vi "test_lidar3.vi"() -> ()   [LabVIEW 2017]
panel:
  out "subarray 2":dbl[][](array[numeric])
  out "subarray 1":dbl[][](array[numeric])
  out "Boucle 2":bool
  out "Boucle 1":bool
  out "output array":dbl[][](array[numeric])
  in  "Array":dbl[][](array[numeric])=[[0.0, 1.0, 2.0, 3.0, 4.0, 355.0, 356.0, 357.0, 358.0, 359.0], [26.0, 12.0, 15.0, 32.0, 27.0, 22.0, 11.0, 23.0, 51.0, 16.0], [0.0, 0.0, 0.0, 0.0, 0.0, 0.0, 0.0, 0.0, 0.0, 0.0]]
  out "Div":dbl
  in  "Alpha 2":i32=8
  out "Nbr a enlever 2":i32
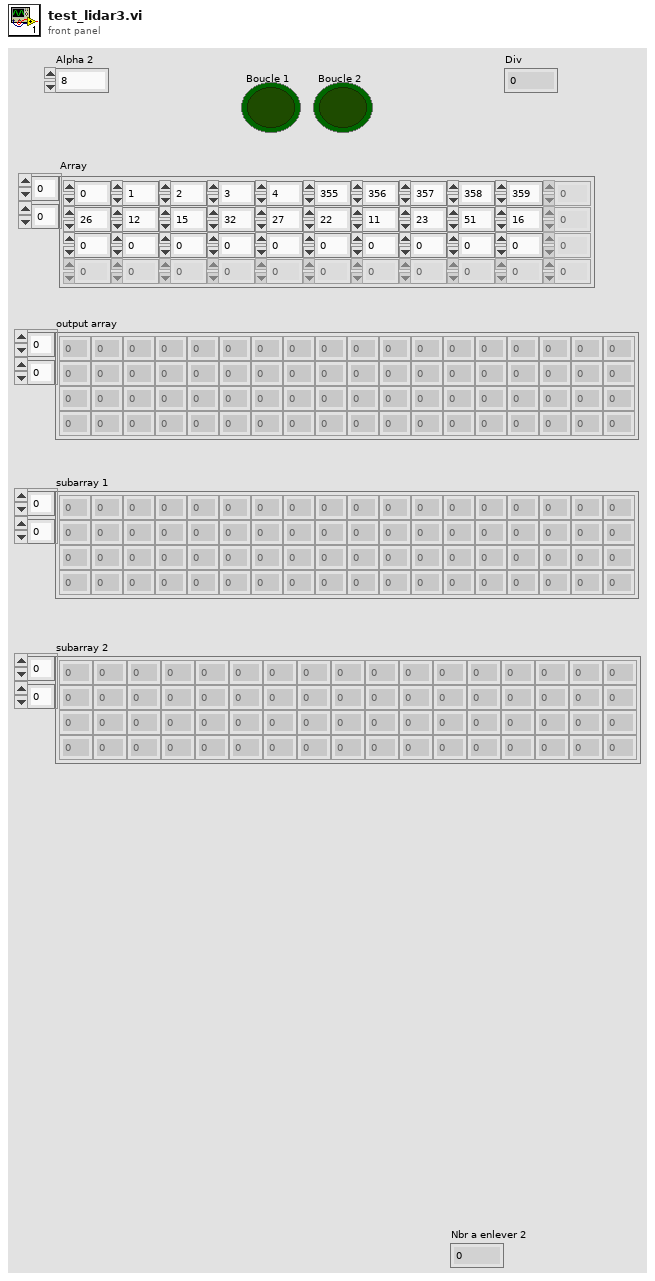
[diagram p1: front panel]
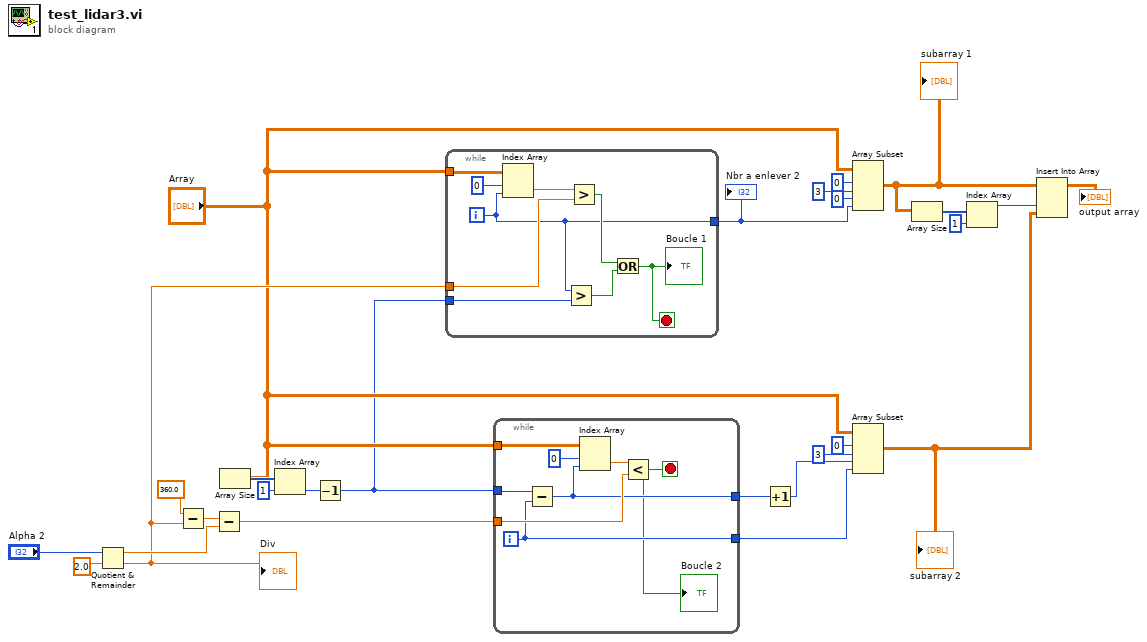
[diagram p0: block diagram]
diagram:
  n1 = Quotient & Remainder(x="Alpha 2", y=2.0) -> (x-y*floor(x/y)=w24:dbl, floor(x/y)=w9:dbl)
  "Div" <- w9
  n2 = Subtract(x=360.0, y=w9) -> (x-y=w26:dbl)
  n3 = Subtract(x=w26, y=w24) -> (x-y=w16:dbl)
  n4 = Array Size(array="Array") -> (size(s)=w19:i32[])
  n5 = Index Array(array=w19, index=1) -> (element=w17:i32)
  n6 = Decrement(x=w17) -> (x-1=w2:i32)
  n7 = while {
    tunnel: "Array" -> [w36]
    tunnel: w9 -> [w34]
    tunnel: [w29] -> w20
    tunnel: w2 -> [w28]
    i -> [w29]
    stop <- w31 stop-if-true
    n8 = Index Array(array=w36, index (row)=0, index (col)=w29) -> (element=w33:dbl)
    n9 = Greater?(x=w29, y=w28) -> (0:w30:bool)
    n10 = Greater?(x=w33, y=w34) -> (0:w32:bool)
    n11 = Or(x=w32, y=w30) -> (x .or. y?=w31:bool)
    "Boucle 1" <- w31
  }
  "Nbr a enlever 2" <- w20
  n12 = while {
    tunnel: "Array" -> [w43]
    tunnel: w2 -> [w42]
    tunnel: w16 -> [w40]
    tunnel: [w39] -> w12
    tunnel: [w38] -> w11
    i -> [w38]
    stop <- w37 stop-if-true
    n13 = Subtract(x=w42, y=w38) -> (x-y=w39:i32)
    n14 = Index Array(array=w43, index (row)=0, index (col)=w39) -> (element=w41:dbl)
    n15 = Less?(x=w41, y=w40) -> (x < y?=w37:bool)
    "Boucle 2" <- w37
  }
  n16 = Increment(x=w12) -> (x+1=w13:i32)
  n17 = Array Subset(array="Array", index (row)=0 ("index"), length (row)=3 ("length"), index (col)=0 ("index"), length (col)=w20) -> (w4:dbl[][])
  "subarray 1" <- w4
  n18 = Array Subset(array="Array", index (row)=0 ("index"), length (row)=3 ("length"), index (col)=w13, length (col)=w11) -> (w1:dbl[][])
  "subarray 2" <- w1
  n19 = Array Size(array=w4) -> (size(s)=w7:i32[])
  n20 = Index Array(array=w7, index=1) -> (element=w5:i32)
  n21 = Insert Into Array(array=w4, index (col)=w5, new element=w1) -> (→"output array":dbl[][])  [unwired: 1 in]
